vi "DMM .vi"(8 "error in (no error)":errorcluster, 9 "Function":u8(ring)=8 items=["DC Voltage", "AC Voltage", "DC Current", "AC Current", "2-Wire Resistance", "4-Wire Resistance", "Frequency", "Period", "None"], 10 "Enum":T1, 11 "VISA resource name":refnum<visa-resource-name>) -> (0 "error out":errorcluster, 3 "Measured":string)   [LabVIEW 2021]
uses:
  DMM_Operation.ctl
  GDM-9052/GDM-9052.lvlib
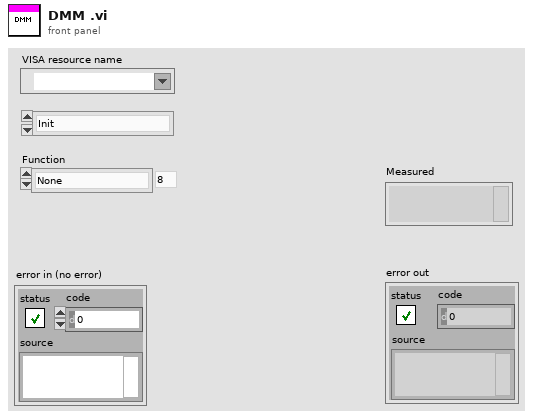
[diagram p1: front panel]
types:
  T1 = typedef "DMM_Operation.ctl" = enum16{"Init", "Configure", "Voltage", "Resistance", "Reset", "Clear", "Close"}
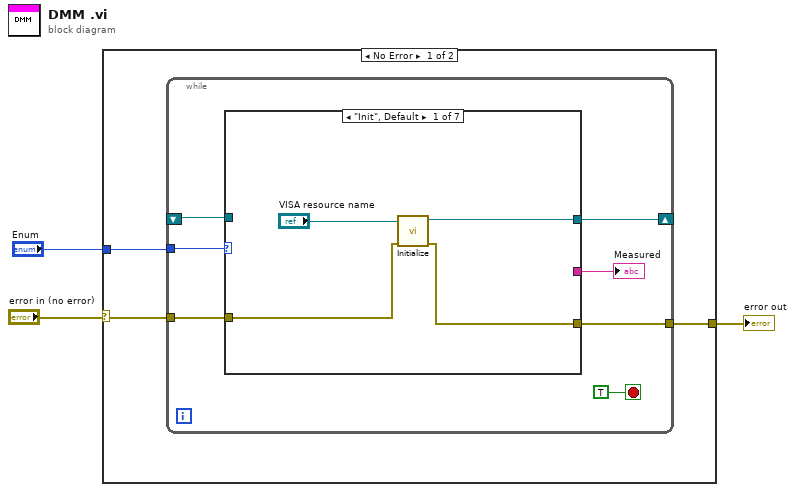
[diagram p0: block diagram]
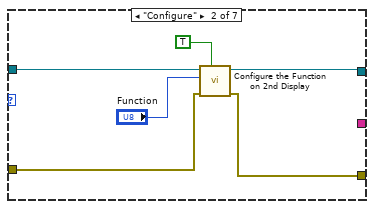
[diagram p2: hidden frame]
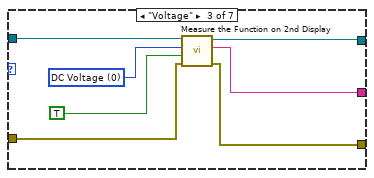
[diagram p3: hidden frame]
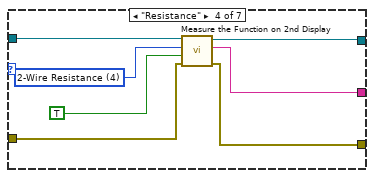
[diagram p4: hidden frame]
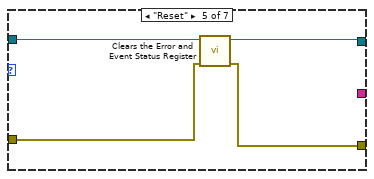
[diagram p5: hidden frame]
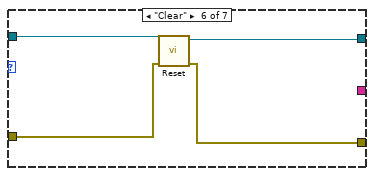
[diagram p6: hidden frame]
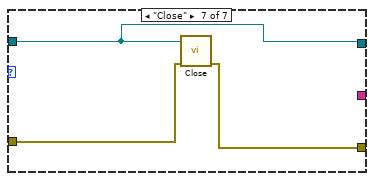
[diagram p7: hidden frame]
diagram:
  n1 = case shown="No Error" "error in (no error)" {
    selector: "error in (no error)" -> [w4 w49]
    tunnel: "Enum" -> [w6 _]
    tunnel: [w5 w49] -> w2
    frame No Error {
      n2 = while {
        tunnel: w6 -> [w13]
        shift-right: [w11] -> _
        shift-left: _ -> [w10]
        tunnel: w4 -> [w8]
        tunnel: [w7] -> w5
        stop <- TRUE stop-if-true
        n3 = case shown="\"Init\", Default" w13 {
          tunnel: [w16 w23 w29 w36 w40 w44 w48] -> w11
          tunnel: w10 -> [_ w22 w30 w37 w41 w45 w48]
          tunnel: [_ _ w26 w33 _ _ _] -> w9
          tunnel: w8 -> [w15 w21 w25 w32 w39 w42 w47]
          tunnel: [w14 w20 w24 w31 w38 w43 w46] -> w7
          frame "Init", Default {
            n4 = call "Initialize.vi"("error in (no error)"=w15, "VISA resource name"="VISA resource name") -> ("error out"=w14:errorcluster, "VISA resource name out"=w16:refnum<visa-resource-name>)  [unwired: 6 in, 2 out]
          }
          frame "Configure" {
            n5 = call "Configure the Function on 2nd Display.vi"("Enable Auto Range"=TRUE, "error in"=w21, "Function"="Function", "VISA resource name"=w22) -> ("error out"=w20:errorcluster, "VISA resource name out"=w23:refnum<visa-resource-name>)  [unwired: 6 in]
          }
          frame "Voltage" {
            w27 = u8 0 items=["DC Voltage", "AC Voltage", "DC Current", "AC Current", "2-Wire Resistance", "4-Wire Resistance", "Frequency", "Period"] ("Function")
            n6 = call "Measure the Function on 2nd Display.vi"("error in"=w25, "Enable Auto Range"=TRUE, "Function"=w27, "VISA resource name"=w30) -> ("error out"=w24:errorcluster, "Return the Value"=w26:string, "VISA resource name out"=w29:refnum<visa-resource-name>)  [unwired: 5 in]
          }
          frame "Resistance" {
            w34 = u8 4 items=["DC Voltage", "AC Voltage", "DC Current", "AC Current", "2-Wire Resistance", "4-Wire Resistance", "Frequency", "Period"] ("Function")
            n7 = call "Measure the Function on 2nd Display.vi"("error in"=w32, "Enable Auto Range"=TRUE, "Function"=w34, "VISA resource name"=w37) -> ("error out"=w31:errorcluster, "Return the Value"=w33:string, "VISA resource name out"=w36:refnum<visa-resource-name>)  [unwired: 5 in]
          }
          frame "Reset" {
            n8 = call "Clears the Error and Event Status Register.vi"("error in (no error)"=w39, "VISA resource name"=w41) -> ("error out"=w38:errorcluster, "VISA resource name out"=w40:refnum<visa-resource-name>)  [unwired: 8 in]
          }
          frame "Clear" {
            n9 = call "Reset.vi"("error in (no error)"=w42, "VISA resource name"=w45) -> ("error out"=w43:errorcluster, "VISA resource name out"=w44:refnum<visa-resource-name>)  [unwired: 8 in]
          }
          frame "Close" {
            n10 = call "Close.vi"("error in (no error)"=w47, "VISA resource name"=w48) -> ("error out"=w46:errorcluster)  [unwired: 9 in]
          }
        }
        "Measured" <- w9
      }
    }
    frame Error {
    }
  }
  "error out" <- w2
